vi "Sound conversion (dbl, mono).vi"(8 "conver rate? (F)":bool, 9 "output rate":enum16{"11025", "22050", "44100"}(ring), 10 "file rate":enum16{"11025", "22050", "44100"}(ring), 11 "sound in":dbl[](array[numeric])) -> (1 "rate out":enum16{"11025", "22050", "44100"}(ring), 3 "sound out":dbl[](array[numeric]))   [LabVIEW 2021]
doc: "::: CalcExpress Toolkit :::\nCopyright (c) 2000-2026 Konstantin Shifershteyn. All rights reserved."
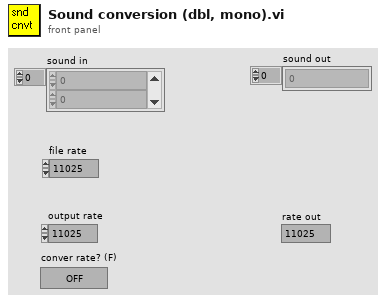
[diagram p1: front panel]
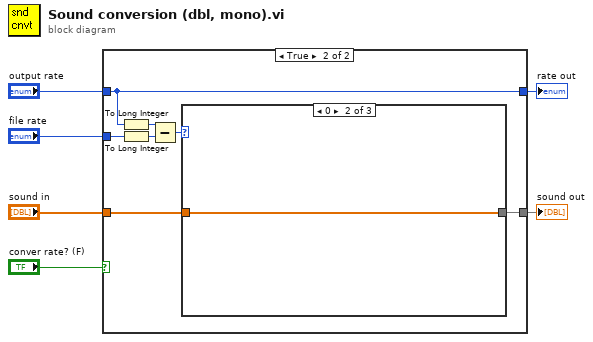
[diagram p0: block diagram]
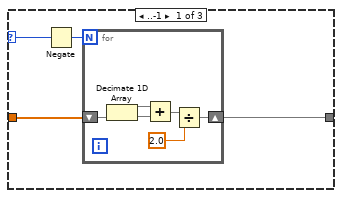
[diagram p3: hidden frame]
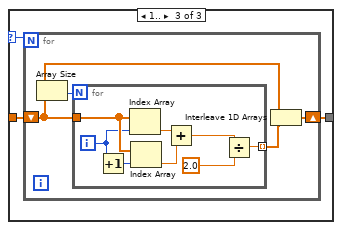
[diagram p4: hidden frame]
diagram:
  n1 = case shown="True" "conver rate? (F)" {
    tunnel: "sound in" -> [w8 w11]
    tunnel: "file rate" -> [w7 w13]
    tunnel: [w8 w10] -> w5
    tunnel: [w7 w9] -> w4
    tunnel: "output rate" -> [_ w9]
    frame False {
    }
    frame True {
      n2 = To Long Integer(number=w9) -> (32bit integer=w14:i32)
      n3 = To Long Integer(number=w13) -> (32bit integer=w15:i32)
      n4 = Subtract(x=w14, y=w15) -> (x-y=w12:i32)
      n5 = case shown="0" w12 {
        selector: w12 -> [w18 _ w28]
        tunnel: w11 -> [w17 w26 w29]
        tunnel: [w16 w26 w27] -> w10
        frame ..-1 {
          n6 = Negate(x=w18) -> (-x=w19:i32)
          n7 = for {
            N: w19 -> [_]
            shift-right: [w20] -> w16
            shift-left: w17 -> [w25]
            n8 = Decimate 1D Array(w25) -> (w24:dbl[], w23:dbl[])
            n9 = Add(x=w24, y=w23) -> (x+y=w22:dbl[])
            n10 = Divide(x=w22, y=2.0) -> (x/y=w20:dbl[])
          }
        }
        frame 0 {
        }
        frame 1.. {
          n11 = for {
            N: w28 -> [_]
            shift-right: [w31] -> w27
            shift-left: w29 -> [w33]
            n12 = Array Size(array=w33) -> (size(s)=w30:i32)
            n13 = for {
              N: w30 -> [_]
              tunnel: w33 -> [w40]
              tunnel: [w36] -> w32 mode=indexing
              i -> [w39]
              n14 = Increment(x=w39) -> (x+1=w41:i32)
              n15 = Index Array(array=w40, index=w39) -> (element=w38:dbl)
              n16 = Index Array(array=w40, index=w41) -> (element=w37:dbl)
              n17 = Add(x=w38, y=w37) -> (x+y=w35:dbl)
              n18 = Divide(x=w35, y=2.0) -> (x/y=w36:dbl)
            }
            n19 = Interleave 1D Arrays(w33, w32) -> (w31:dbl[])
          }
        }
      }
    }
  }
  "sound out" <- w5
  "rate out" <- w4
